vi "Merge Image Manager.vi"(7 "Calling VI Ref":refnum<vi>) -> ()   [LabVIEW 2016]
uses:
  Merge Image Type Defs/Merge Image - Image Control.ctl
  <vilib>/Utility/miscctls.llb/LVPointTypeDef.ctl
  <vilib>/vision/Image Controls.llb/IMAQ Image.ctl
  Merge Image Type Defs/Merge Image - Notifier Type.ctl
  Merge Image Type Defs/Merge Image - Actions.ctl
  Merge Image Type Defs/Merge Image - Last Used Save Type.ctl
  <vilib>/vision/NI_Vision_Development_Module.lvlib
panel:
  in  "Zero All":bool
  out "Overlay Error":errorcluster
  in  "Load":bool
  in  "Save":bool
  in  "Update Rate (ms)":i32=50
  in  "Merge Visible":bool
  in  "Hold Blue":bool
  in  "Hold Green":bool
  in  "Hold Red":bool
  in  "Blue LUT":cluster{"Blue Min (%)":i32, "Blue Max (%)":i32}={"Blue Min (%)"=0, "Blue Max (%)"=100} {"Blue Max (%)" max=100; "Blue Min (%)" max=100}
  in  "Green LUT":T1={"Green Min (%)"=0, "Green Max (%)"=100} {"Green Max (%)" max=100; "Green Min (%)" max=100}
  in  "Red LUT":cluster{"Red Min (%)":i32, "Red Max (%)":i32}={"Red Min (%)"=0, "Red Max (%)"=100} {"Red Max (%)" max=100; "Red Min (%)" max=100}
  in  "Blue Image":T2 {"Rotation (°)" format="%#.2f"; "Image" items=["None", "Image 01", "Image 02", "Merge Image"]}
  in  "Green Image":T2 {"Rotation (°)" format="%#.2f"; "Image" items=["None", "Image 01", "Image 02", "Merge Image"]}
  in  "Red Image":T2 {"Rotation (°)" format="%#.2f"; "Image" items=["None", "Image 01", "Image 02", "Merge Image"]}
  in  "Quit":bool
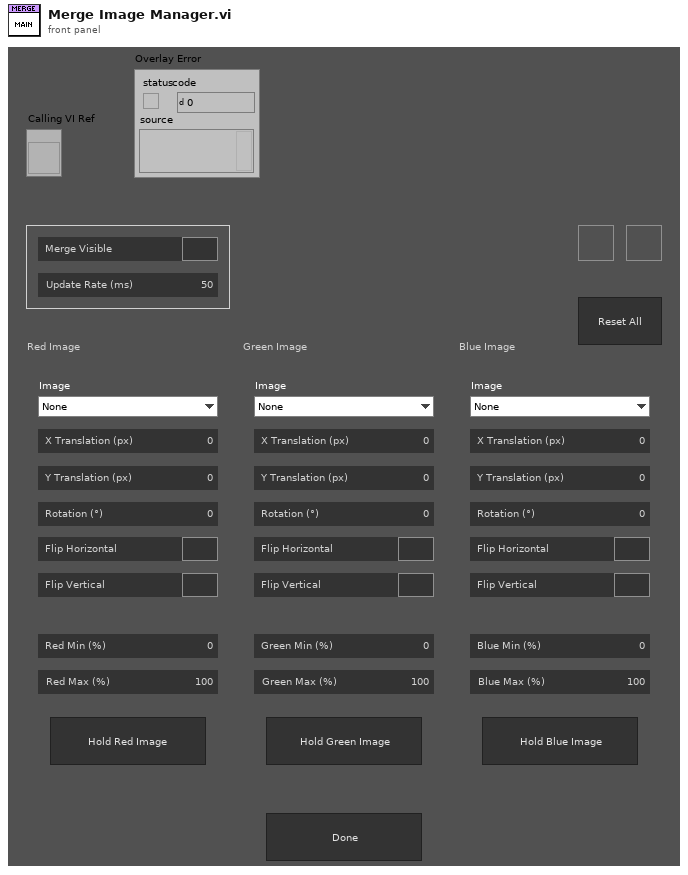
[diagram p1: front panel]
types:
  T1 = cluster{"Green Min (%)":i32, "Green Max (%)":i32}
  T2 = typedef "Merge Image - Image Control.ctl" = cluster{"Image":i32, "X Translation (px)":i32, "Y Translation (px)":i32, "Rotation (°)":sgl, "Flip Horizontal":bool, "Flip Vertical":bool}
  T3 = typedef "Merge Image - Last Used Save Type.ctl" = cluster{"Merge Contols":T2[], "LUT Controls":cluster{"Red Min (%)":i32, "Red Max (%)":i32}[]}
  T4 = typedef "Image Type" = u32
  T5 = typedef "Merge Image - Actions.ctl" = enum16{"Timeout", "Update Image Source", "Update LUTs", "Quit"}
  T6 = typedef "Merge Image - Notifier Type.ctl" = cluster{"Actions":T5, "Merge Contols":T2[], "LUT Controls":cluster{"Red Min (%)":i32, "Red Max (%)":i32}[]}
  T7 = typedef "IMAQ Image.ctl" = refnum<image>
  T8 = enum16{"Always On", "Always Off", "Off While Running"}
  T9 = typedef "LVPointTypeDef.ctl" = cluster{"Horizontal":i16, "Vertical":i16}
  T10 = typedef "LVRectTypeDef.ctl" = cluster{"Left":i16, "Top":i16, "Right":i16, "Bottom":i16}
  T11 = typedef "LVBoundsTypeDef.ctl" = cluster{"Width":u32, "Height":u32}
  T12 = enum32{"Invalid", "Standard", "Closed", "Hidden", "Minimized", "Maximized"}
  T13 = enum32{"Invalid", "Default", "Floating", "Floating/Auto-Hide", "Modal"}
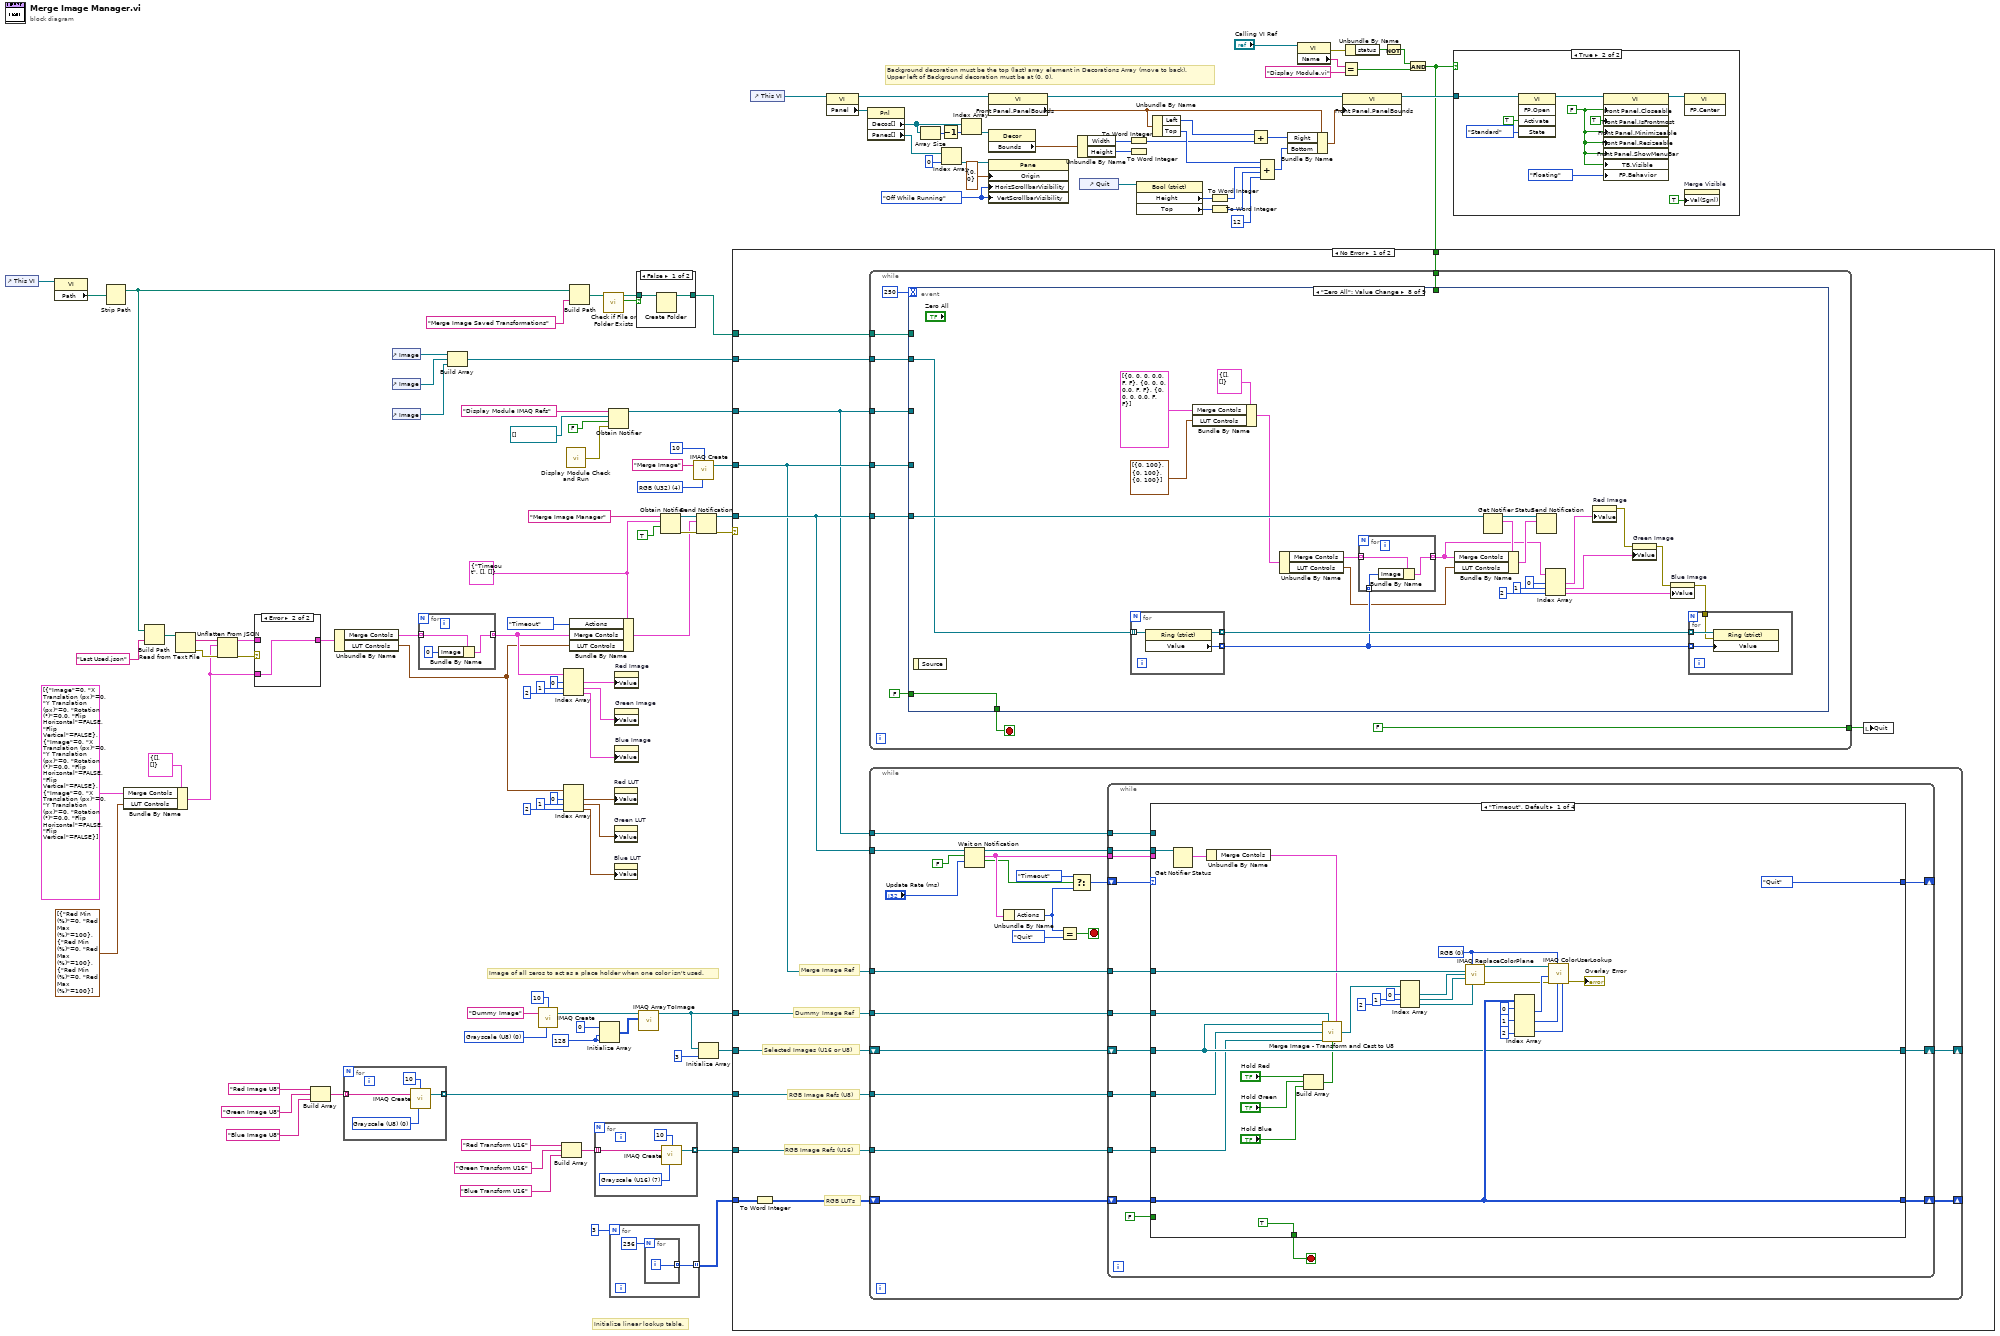
[diagram p0: block diagram]
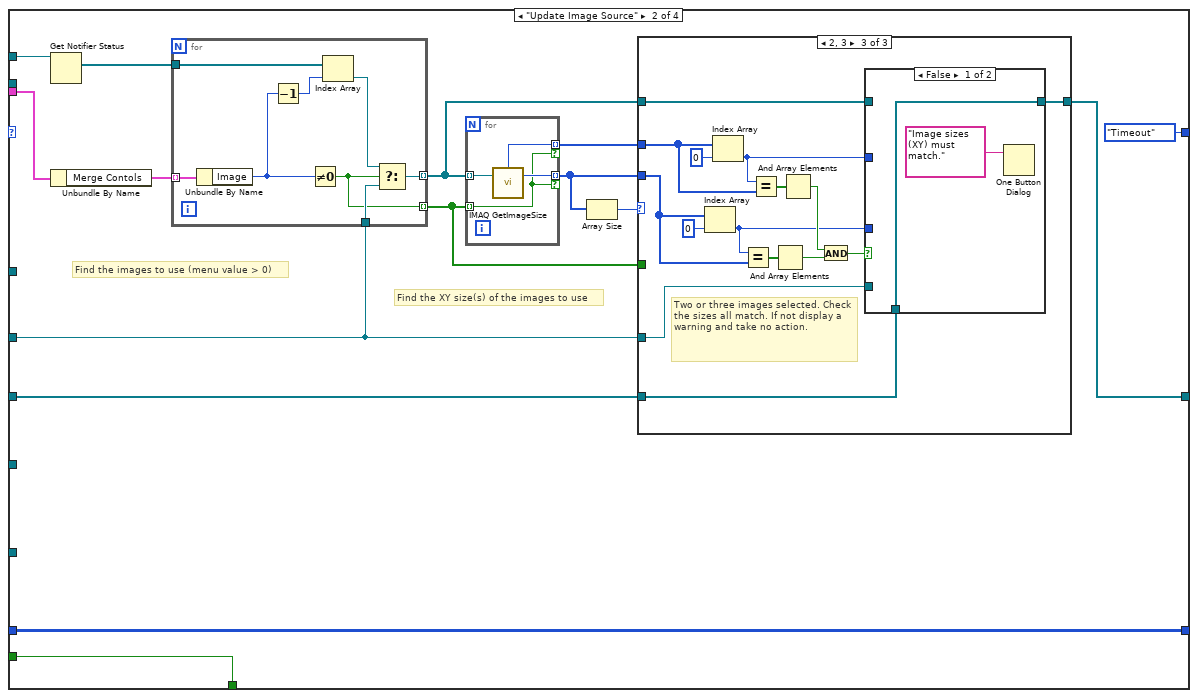
[diagram p5: hidden frame]
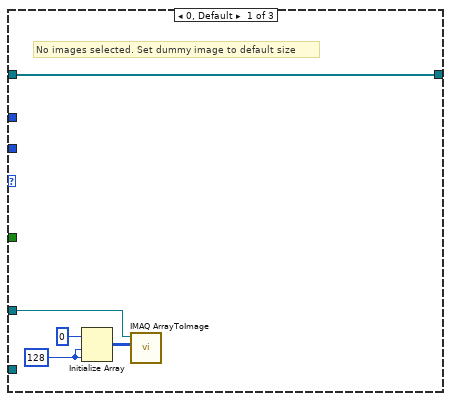
[diagram p6: hidden frame]
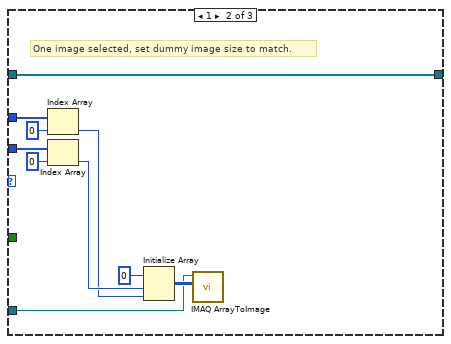
[diagram p7: hidden frame]
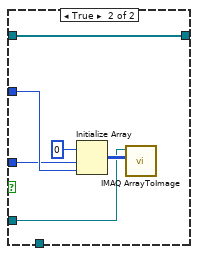
[diagram p8: hidden frame]
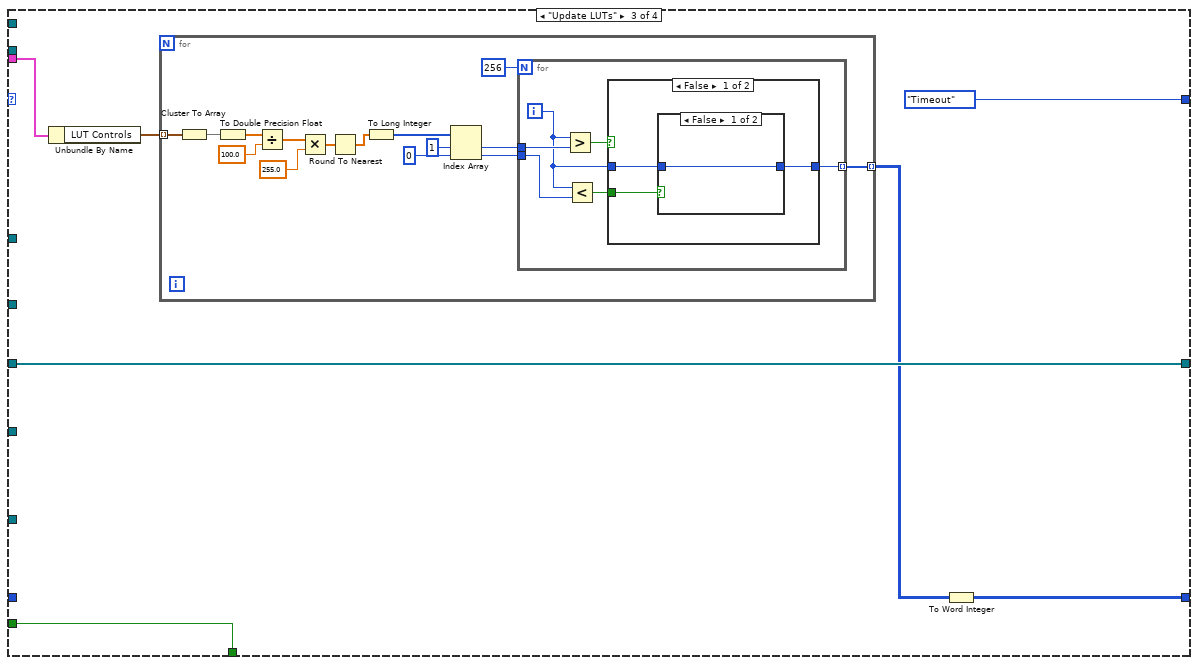
[diagram p9: hidden frame]
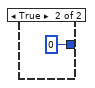
[diagram p10: hidden frame]
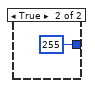
[diagram p11: hidden frame]
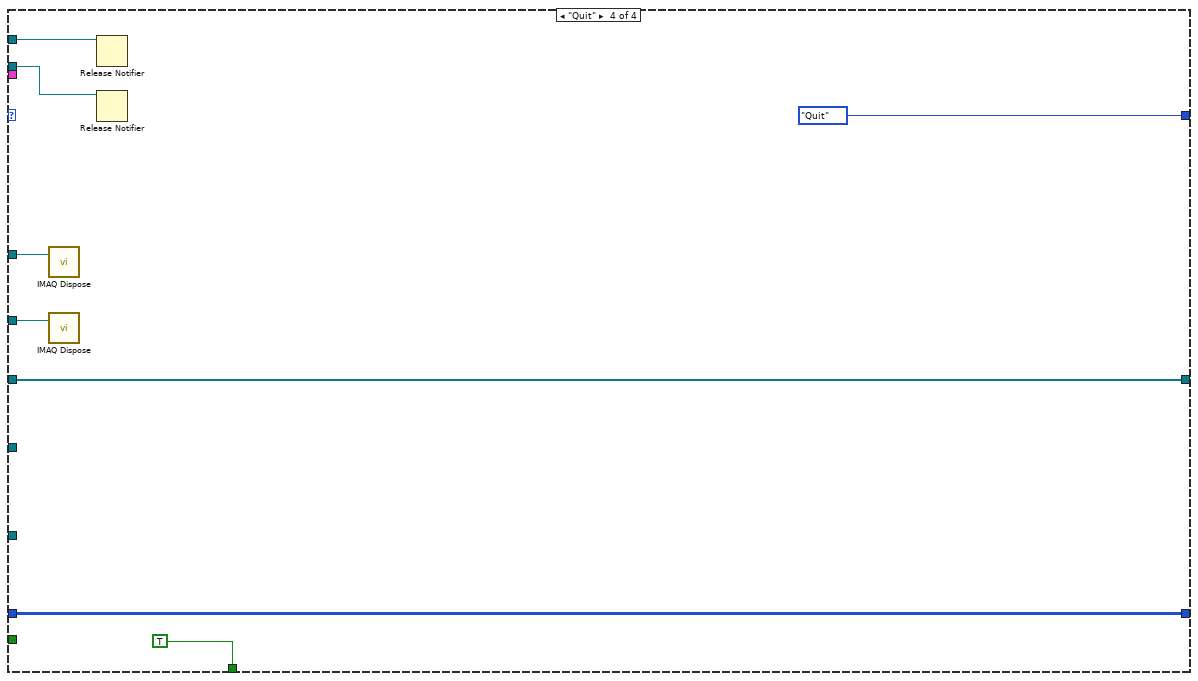
[diagram p12: hidden frame]
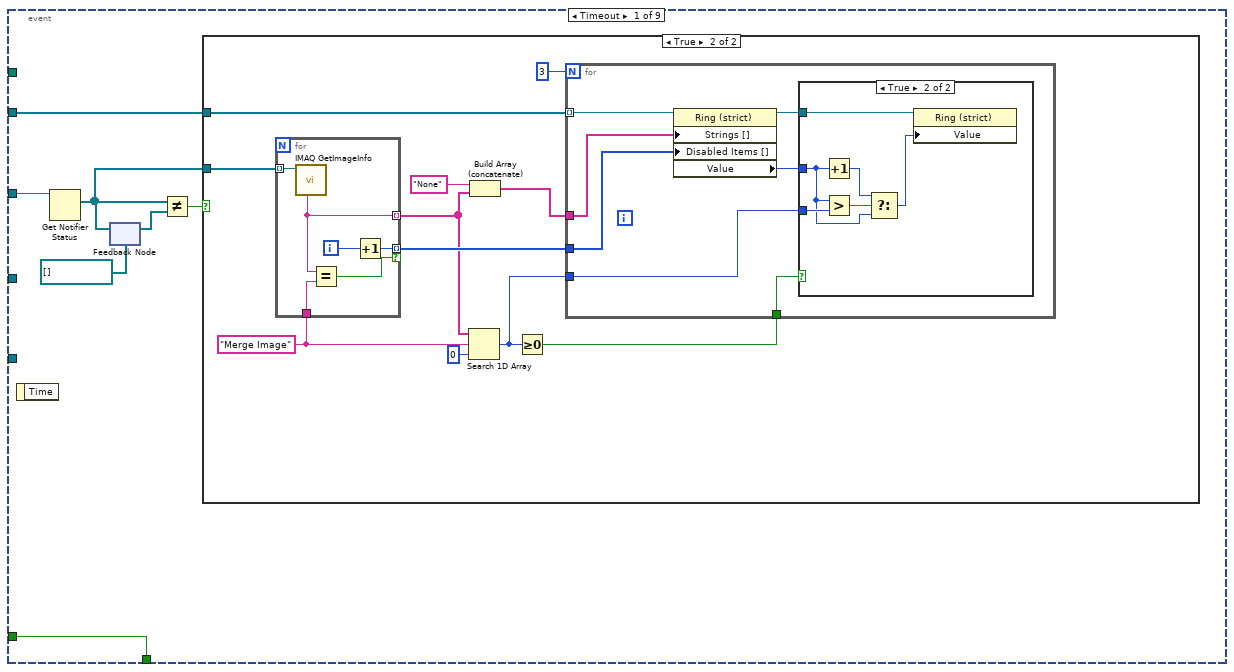
[diagram p13: hidden frame]
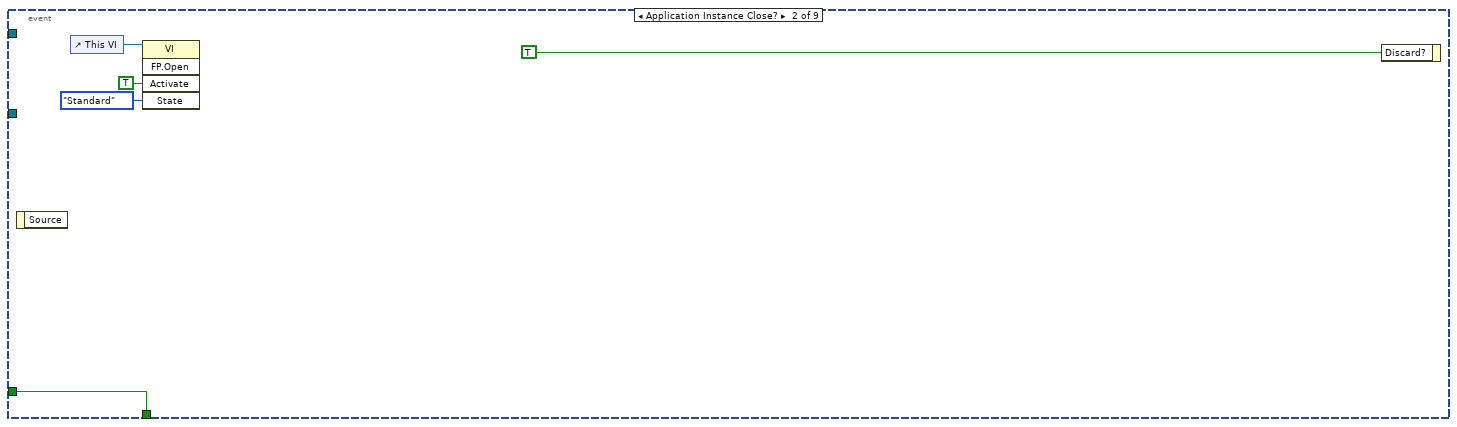
[diagram p16: hidden frame]
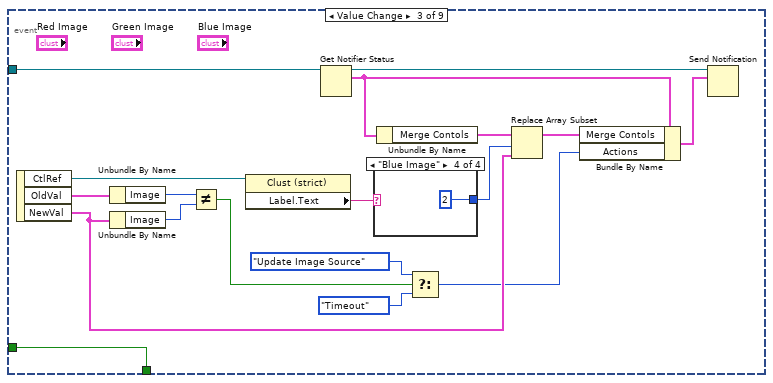
[diagram p17: hidden frame]
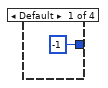
[diagram p18: hidden frame]
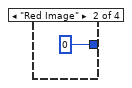
[diagram p19: hidden frame]
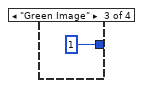
[diagram p20: hidden frame]
diagram:
  w53 = 128 ("dimension size")
  w58 = T4 0 items=["Grayscale (U8)", "Grayscale (I16)", "Grayscale (SGL)", "Complex (CSG)", "RGB (U32)", "HSL (U32)", "RGB (U64)", "Grayscale (U16)"] ("Image Type")
  w62 = T6 {"Actions"=enum."Timeout", "Merge Contols"=[], "LUT Controls"=[]} ("Merge Image Notifier Type")
  w71 = T4 4 items=["Grayscale (U8)", "Grayscale (I16)", "Grayscale (SGL)", "Complex (CSG)", "RGB (U32)", "HSL (U32)", "RGB (U64)", "Grayscale (U16)"] ("Image Type")
  w99 = T8."Off While Running" ("Vertical Scrollbar Visibility")
  # "Image of all zeros to act as a place holder when one color isn't used."
  # "Initialize linear lookup table."
  # "Background decoration must be the top (last) array element in Decorations Array (move to back).\nUpper left of Background decoration must be at (0, 0)."
  n1 = control-ref of="This VI"() -> (w83:refnum<vi>)
  n2 = property class="VI"(reference=w83) -> ("Path"=w82:path)  [unwired: 1 in, 2 out]
  n3 = Strip Path(path=w82) -> (stripped path=w26:path)  [unwired: 1 out]
  n4 = Bundle By Name(cluster=T3 {"Merge Contols"=[], "LUT Controls"=[]} ("Merge Image Last Used Type"), "Merge Contols"=T2[] [{"Image"=0, "X Translation (px)"=0, "Y Translation (px)"=0, "Rotation (°)"=0.0, "Flip Horizontal"=FALSE, "Flip Vertical"=FALSE}, {"Image"=0, "X Translation (px)"=0, "Y Translation (px)"=0, "Rotation (°)"=0.0, "Flip Horizontal"=FALSE, "Flip Vertical"=FALSE}, {"Image"=0, "X Translation (px)"=0, "Y Translation (px)"=0, "Rotation (°)"=0.0, "Flip Horizontal"=FALSE, "Flip Vertical"=FALSE}], "LUT Controls"=cluster{"Red Min (%)":i32, "Red Max (%)":i32}[] [{"Red Min (%)"=0, "Red Max (%)"=100}, {"Red Min (%)"=0, "Red Max (%)"=100}, {"Red Min (%)"=0, "Red Max (%)"=100}]) -> (w5:T3)
  n5 = Build Path(base path=w26, name or relative path="Last Used.json") -> (appended path=w25:path)
  n6 = Read from Text File(file (use dialog)=w25) -> (text=w24:string, error out=w23:errorcluster)  [unwired: 3 in, 2 out]
  n7 = Unflatten From JSON(JSON string=w24, type and defaults=w5, error in (no error)=w23) -> (value=w21:T3, error out=w22:errorcluster)  [unwired: 4 in]
  n8 = case shown="Error" w22 {
    tunnel: w21 -> [w117 _]
    tunnel: [w117 w118] -> w4
    tunnel: w5 -> [_ w118]
    frame No Error {
    }
    frame Error {
    }
  }
  n9 = Build Array("Red Image U8" ("Image Name"), "Green Image U8" ("Image Name"), "Blue Image U8" ("Image Name")) -> (w47:string[])
  n10 = Unbundle By Name(w4) -> ("Merge Contols"=w3:T2[], "LUT Controls"=w1:cluster{"Red Min (%)":i32, "Red Max (%)":i32}[])
  n11 = for {
    tunnel: w47 -> [w120] mode=indexing
    tunnel: [w119] -> w46 mode=indexing
    w121 = T4 0 items=["Grayscale (U8)", "Grayscale (I16)", "Grayscale (SGL)", "Complex (CSG)", "RGB (U32)", "HSL (U32)", "RGB (U64)", "Grayscale (U16)"] ("Image Type")
    n12 = call "IMAQ Create"("Border Size"=10, "Image Name"=w120, "Image Type"=w121) -> ("New Image"=w119:T7)  [unwired: 2 in, 1 out]
  }
  n13 = control-ref of="Image"() -> (w67:refnum<vi>)
  n14 = control-ref of="Image"() -> (w65:refnum<vi>)
  n15 = control-ref of="Image"() -> (w66:refnum<vi>)
  n16 = for {
    tunnel: w3 -> [w125] mode=indexing
    tunnel: [w123] -> w2 mode=indexing
    n17 = Bundle By Name(cluster=w125, "Image"=0) -> (w123:T2)
  }
  n18 = Build Array(w67, w65, w66) -> (w64:refnum<vi>[])
  n19 = call "IMAQ Create"("Border Size"=10, "Image Name"="Dummy Image", "Image Type"=w58) -> ("New Image"=w59:T7)  [unwired: 2 in, 1 out]
  n20 = Build Array("Red Transform U16" ("Image Name"), "Green Transform U16" ("Image Name"), "Blue Transform U16" ("Image Name")) -> (w42:string[])
  n21 = Index Array(array=w2, index #1=0 ("index"), index #2=1 ("index"), index #3=2 ("index")) -> (element #1=w17:T2, element #2=w15:T2, element #3=w16:T2)
  n22 = Index Array(array=w1, index #1=0 ("index"), index #2=1 ("index"), index #3=2 ("index")) -> (element #1=w11:cluster{"Red Min (%)":i32, "Red Max (%)":i32}, element #2=w9:cluster{"Red Min (%)":i32, "Red Max (%)":i32}, element #3=w10:cluster{"Red Min (%)":i32, "Red Max (%)":i32})
  n23 = call "Display Module Check and Run.vi"() -> ("Error"=w63:errorcluster)  [unwired: 15 in]
  n24 = Bundle By Name(cluster=w62, "Actions"=Merge_Image_-_Actions."Timeout", "Merge Contols"=w2, "LUT Controls"=w1) -> (w60:T6)
  n25 = Build Path(base path=w26, name or relative path="Merge Image Saved Transformations") -> (appended path=w80:path)
  n26 = for {
    tunnel: w42 -> [w127] mode=indexing
    tunnel: [w126] -> w38 mode=indexing
    w128 = T4 7 items=["Grayscale (U8)", "Grayscale (I16)", "Grayscale (SGL)", "Complex (CSG)", "RGB (U32)", "HSL (U32)", "RGB (U64)", "Grayscale (U16)"] ("Image Type")
    n27 = call "IMAQ Create"("Border Size"=10, "Image Name"=w127, "Image Type"=w128) -> ("New Image"=w126:T7)  [unwired: 2 in, 1 out]
  }
  n28 = Initialize Array(u8 0 ("element"), w53, w53) -> (w54:u8[][])
  n29 = call <vilib>:"Check if File or Folder Exists.vi"("path"=w80) -> ("file or folder exists?"=w79:bool, "dup path"=w78:path)  [unwired: 8 in, 1 out]
  n30 = Obtain Notifier(name (unnamed)="Display Module IMAQ Refs", notification data type=T7[] [], create if not found? (T)=FALSE, error in (no error)=w63) -> (notifier out=w68:refnum<notifier>)  [unwired: 2 out]
  n31 = for {
    N: 3 -> [_]
    tunnel: [w130] -> w51 mode=indexing
    n32 = for {
      N: 256 -> [_]
      tunnel: [w132] -> w130 mode=indexing
      i -> [w132]
    }
  }
  n33 = property on="Red LUT" class="Clust (strict)"("Value"=w11) -> ()  [unwired: 2 in, 2 out]
  n34 = property on="Green LUT" class="Clust (strict)"("Value"=w9) -> ()  [unwired: 2 in, 2 out]
  n35 = property on="Blue LUT" class="Clust (strict)"("Value"=w10) -> ()  [unwired: 2 in, 2 out]
  n36 = property on="Red Image" class="Clust (strict)"("Value"=w17) -> ()  [unwired: 2 in, 2 out]
  n37 = property on="Green Image" class="Clust (strict)"("Value"=w15) -> ()  [unwired: 2 in, 2 out]
  n38 = property on="Blue Image" class="Clust (strict)"("Value"=w16) -> ()  [unwired: 2 in, 2 out]
  n39 = case shown="False" w79 {
    tunnel: w78 -> [w134 w135]
    tunnel: [w133 w135] -> w37
    frame False {
      n40 = Create Folder(path (use dialog)=w134) -> (created path=w133:path)  [unwired: 2 in, 2 out]
    }
    frame True {
    }
  }
  n41 = call "IMAQ ArrayToImage"("Image Pixels (U8)"=w54, "Image"=w59) -> ("Image Out"=w43:T7)  [unwired: 8 in, 1 out]
  n42 = Obtain Notifier(name (unnamed)="Merge Image Manager", notification data type=w62, create if not found? (T)=TRUE) -> (notifier out=w85:refnum<notifier>, error out=w77:errorcluster)  [unwired: 1 in, 1 out]
  n43 = call "IMAQ Create"("Border Size"=10, "Image Name"="Merge Image", "Image Type"=w71) -> ("New Image"=w69:T7)  [unwired: 2 in, 1 out]
  n44 = Send Notification(notification=w60, notifier=w85, error in (no error)=w77) -> (notifier out=w84:refnum<notifier>, error out=w76:errorcluster)
  n45 = Initialize Array(w43, 3 ("dimension size")) -> (w44:T7[])
  n46 = control-ref of="This VI"() -> (w91:refnum<vi>)
  n47 = property class="VI"(reference=w91) -> (reference out=w100:refnum<vi>, "Panel"=w92:refnum<vi>)  [unwired: 1 in, 1 out]
  n48 = property class="Pnl"(reference=w92) -> ("Decos[]"=w90:refnum<vi>[], "Panes[]"=w96:refnum<vi>[])  [unwired: 1 in, 2 out]
  n49 = Array Size(array=w90) -> (size(s)=w88:i32)
  n50 = Decrement(x=w88) -> (x-1=w89:i32)
  n51 = Index Array(array=w96, index=0) -> (element=w95:refnum<vi>)
  n52 = Index Array(array=w90, index=w89) -> (element=w98:refnum<vi>)
  n53 = property class="VI"(reference=w100) -> (reference out=w102:refnum<vi>, "Front Panel.PanelBounds"=w103:T10)  [unwired: 1 in, 1 out]
  n54 = property class="Decor"(reference=w98) -> ("Bounds"=w101:T11)  [unwired: 1 in, 2 out]
  n55 = property class="Pane"(reference=w95, "Origin"=T9 {"Horizontal"=0, "Vertical"=0}, "HorizScrollbarVisibility"=w99, "VertScrollbarVisibility"=w99) -> ()  [unwired: 1 in, 2 out]
  n56 = Unbundle By Name(w101) -> ("Width"=w106:u32, "Height"=w109:u32)
  n57 = control-ref of="Quit"() -> (w93:refnum<vi>)
  n58 = To Word Integer(number=w106) -> (16bit integer=w108:i16)
  n59 = To Word Integer(number=w109) -> ()  [unwired: 1 out]
  n60 = property class="Bool (strict)"(reference=w93) -> ("Height"=w111:u32, "Top"=w112:i32)  [unwired: 1 in, 2 out]
  n61 = Unbundle By Name(w103) -> ("Left"=w105:i16, "Top"=w116:i16)
  n62 = To Word Integer(number=w111) -> (16bit integer=w114:i16)
  n63 = To Word Integer(number=w112) -> (16bit integer=w115:i16)
  n64 = Add(x=w105, y=w108) -> (x+y=w107:i16)
  n65 = Compound Arithmetic op=ADD(w116, w114, w115, i16 12 ("y")) -> (w110:i16)
  n66 = Bundle By Name(cluster=w103, "Right"=w107, "Bottom"=w110) -> (w104:T10)
  n67 = property class="VI"(reference="Calling VI Ref") -> (error out=w32:errorcluster, "Name"=w35:string)  [unwired: 1 in, 1 out]
  n68 = Equal?(x=w35, y="Display Module.vi") -> (x = y?=w29:bool)
  n69 = property class="VI"(reference=w102, "Front Panel.PanelBounds"=w104) -> (reference out=w33:refnum<vi>)  [unwired: 1 in, 1 out]
  n70 = Unbundle By Name(w32) -> ("status"=w31:bool)
  n71 = Not(x=w31) -> (.not. x?=w30:bool)
  n72 = And(x=w30, y=w29) -> (x .and. y?=w28:bool)
  n73 = case shown="No Error" w76 {
    selector: w76 -> [_ w566]
    tunnel: w84 -> [w147 w568]
    tunnel: w69 -> [w143 w567]
    tunnel: w68 -> [w142 w569]
    tunnel: w64 -> [w146 _]
    tunnel: w43 -> [w145 _]
    tunnel: w46 -> [w141 _]
    tunnel: w51 -> [w144 _]
    tunnel: w44 -> [w140 _]
    tunnel: w38 -> [w139 _]
    tunnel: w37 -> [w137 _]
    tunnel: w28 -> [w136 _]
    frame No Error {
      # "RGB Image Refs (U16)"
      # "Selected Images (U16 or U8)"
      # "Merge Image Ref"
      # "Dummy Image Ref"
      # "RGB Image Refs (U8)"
      # "RGB LUTs"
      n74 = To Word Integer(number=w144) -> (16bit integer=w138:i16[][])
      n75 = while {
        tunnel: w147 -> [w330]
        tunnel: [FALSE] -> w148
        tunnel: w143 -> [w328]
        tunnel: w142 -> [w327]
        tunnel: w146 -> [w326]
        tunnel: w137 -> [w324]
        tunnel: w136 -> [w323]
        stop <- w331 stop-if-true
        n76 = event shown="[7] \"Zero All\": Value Change" {
          selector: _ -> [_ _ _ _ _ _ _ _ _]
          dyn-events: _ -> [_ _ _ _ _ _ _ _ _]
          timeout: 250 -> [_ _ _ _ _ _ _ _ _]
          tunnel: FALSE -> [w339 w373 w392 w410 w425 w466 w484 w536 _]
          tunnel: [w339 w373 w392 w410 w425 w466 w484 w536 w562] -> w331
          tunnel: w330 -> [_ _ w391 w409 _ w465 w475 w535 w561]
          tunnel: w328 -> [_ _ _ _ w417 _ _ _ _]
          tunnel: w327 -> [w338 _ _ _ w416 _ _ _ _]
          tunnel: w326 -> [w334 _ _ _ w415 _ w472 w534 _]
          tunnel: w324 -> [_ _ _ _ _ w463 w479 _ _]
          tunnel: w323 -> [_ _ _ _ _ _ _ _ w557]
          event Timeout {
            n77 = event-data() -> ()  [unwired: 1 in, 1 out]
            n78 = Get Notifier Status(notifier=w338) -> (current notification=w333:T7[])  [unwired: 1 in, 4 out]
            n79 = feedback-in #1(w333) -> ()
            n80 = feedback #1(T7[] []) -> (w336:T7[])
            n81 = Not Equal?(x=w333, y=w336) -> (x != y?=w335:bool)
            n82 = case shown="True" w335 {
              tunnel: w334 -> [_ w349]
              tunnel: w333 -> [_ w350]
              frame False {
              }
              frame True {
                w343 = "Merge Image" ("Image Name")
                n83 = for {
                  tunnel: w350 -> [w369] mode=indexing
                  tunnel: [w368] -> w344 mode=indexing
                  tunnel: [w367] -> w345 mode=indexing if=w365
                  tunnel: w343 -> [w364]
                  i -> [w366]
                  n84 = call "IMAQ GetImageInfo"("Image"=w369) -> ("Image Name"=w368:string)  [unwired: 3 in, 7 out]
                  n85 = Equal?(x=w368, y=w364) -> (x = y?=w365:bool)
                  n86 = Increment(x=w366) -> (x+1=w367:i32)
                }
                n87 = Search 1D Array(1D array=w344, element=w343, start index (0)=0) -> (index of element=w340:i32)
                n88 = Build Array (concatenate)("None", w344) -> (w347:string[])
                n89 = Greater Or Equal To 0?(x=w340) -> (x >= 0?=w341:bool)
                n90 = for {
                  N: 3 -> [_]
                  tunnel: w349 -> [w357] mode=indexing
                  tunnel: w347 -> [w356]
                  tunnel: w345 -> [w355]
                  tunnel: w341 -> [w352]
                  tunnel: w340 -> [w351]
                  n91 = property class="Ring (strict)"(reference=w357, "Strings []"=w356, "Disabled Items []"=w355) -> (reference out=w354:refnum<vi>, "Value"=w353:i32)  [unwired: 1 in, 1 out]
                  n92 = case shown="True" w352 {
                    tunnel: w354 -> [_ w363]
                    tunnel: w353 -> [_ w358]
                    tunnel: w351 -> [_ w362]
                    frame False {
                    }
                    frame True {
                      n93 = Increment(x=w358) -> (x+1=w360:i32)
                      n94 = Greater?(x=w358, y=w362) -> (0:w361:bool)
                      n95 = Select(t=w360, s=w361, f=w358) -> (s? t:f=w359:i32)
                      n96 = property class="Ring (strict)"(reference=w363, "Value"=w359) -> ()  [unwired: 1 in, 2 out]
                    }
                  }
                }
              }
            }
          }
          event Application Instance Close? {
            n97 = event-data() -> ()  [unwired: 1 in, 1 out]
            n98 = control-ref of="This VI"() -> (w370:refnum<vi>)
            n99 = invoke class="VI" method="FP.Open"(reference=w370, "Activate"=TRUE ("Activate?"), "State"=T12."Standard") -> ()  [unwired: 2 in, 5 out]
            n100 = event-data("Discard?"=TRUE) -> ()  [unwired: 1 in, 1 out]
          }
          event Value Change {
            n101 = event-data() -> ("CtlRef"=w389:refnum<vi>, "OldVal"=w382:T2, "NewVal"=w379:T2)  [unwired: 1 in]
            n102 = Unbundle By Name(w382) -> ("Image"=w381:i32)
            n103 = Unbundle By Name(w379) -> ("Image"=w380:i32)
            n104 = Not Equal?(x=w381, y=w380) -> (x != y?=w378:bool)
            n105 = property class="Clust (strict)"(reference=w389) -> ("Label.Text"=w388:string)  [unwired: 1 in, 2 out]
            n106 = Get Notifier Status(notifier=w391) -> (notifier out=w390:refnum<notifier>, current notification=w383:T6)  [unwired: 1 in, 3 out]
            n107 = case shown="\"Blue Image\"" w388 {
              tunnel: [-1 0 1 2] -> w386
              frame Default {
              }
              frame "Red Image" {
              }
              frame "Green Image" {
              }
              frame "Blue Image" {
              }
            }
            n108 = Unbundle By Name(w383) -> ("Merge Contols"=w387:T2[])
            n109 = Select(t=Merge_Image_-_Actions."Update Image Source" ("Actions"), s=w378, f=Merge_Image_-_Actions."Timeout" ("Actions")) -> (s? t:f=w375:T5)
            n110 = Replace Array Subset(array=w387, new element=w379, index=w386) -> (w385:T2[])
            n111 = Bundle By Name(cluster=w383, "Merge Contols"=w385, "Actions"=w375) -> (w384:T6)
            n112 = Send Notification(notification=w384, notifier=w390) -> ()  [unwired: 1 in, 2 out]
          }
          event "Red LUT", "Green LUT", "Blue LUT": Value Change {
            n113 = event-data() -> ("NewVal"=w399:variant, "CtlRef"=w400:refnum<vi>)  [unwired: 1 in]
            n114 = Variant To Data(type=cluster{"Red Min (%)":u16, "Red Max (%)":u16} {"Red Min (%)"=0, "Red Max (%)"=100} ("LUT Controls"), Variant=w399) -> (data=w397:cluster{"Red Min (%)":u16, "Red Max (%)":u16})  [unwired: 1 in, 1 out]
            n115 = property class="Clust (strict)"(reference=w400) -> ("Label.Text"=w407:string)  [unwired: 1 in, 2 out]
            n116 = Get Notifier Status(notifier=w409) -> (notifier out=w408:refnum<notifier>, current notification=w401:T6)  [unwired: 1 in, 3 out]
            n117 = case shown="\"Red LUT\"" w407 {
              tunnel: [-1 0 1 2] -> w405
              frame Default {
              }
              frame "Red LUT" {
              }
              frame "Green LUT" {
              }
              frame "Blue LUT" {
              }
            }
            n118 = Unbundle By Name(w401) -> ("LUT Controls"=w406:cluster{"Red Min (%)":i32, "Red Max (%)":i32}[])
            n119 = Replace Array Subset(array=w406, new element=w397, index=w405) -> (w404:cluster{"Red Min (%)":i32, "Red Max (%)":i32}[])
            n120 = Bundle By Name(cluster=w401, "Actions"=Merge_Image_-_Actions."Update LUTs", "LUT Controls"=w404) -> (w402:T6)
            n121 = Send Notification(notification=w402, notifier=w408) -> ()  [unwired: 1 in, 2 out]
          }
          event "Merge Visible": Value Change {
            n122 = event-data() -> ("NewVal"=w418:bool)  [unwired: 1 in]
            n123 = Get Notifier Status(notifier=w416) -> (notifier out=w424:refnum<notifier>, current notification=w422:T7[], error out=w423:errorcluster)  [unwired: 1 in, 2 out]
            n124 = case shown="False" w418 {
              tunnel: w424 -> [w434 w451]
              tunnel: w423 -> [w432 w450]
              tunnel: w422 -> [w431 w449]
              tunnel: [w433 w447] -> w419
              tunnel: [w434 w451] -> w421
              tunnel: [w432 w450] -> w420
              tunnel: w417 -> [w430 w448]
              tunnel: w415 -> [w427 _]
              frame False {
                n125 = Search 1D Array(1D array=w431, element=w430, start index (0)=0) -> (index of element=w426:i32)
                n126 = Greater Or Equal To 0?(x=w426) -> (x >= 0?=w428:bool)
                n127 = case shown="True" w428 {
                  tunnel: w426 -> [_ w445]
                  tunnel: w431 -> [w442 w444]
                  tunnel: [w442 w443] -> w433
                  frame False {
                  }
                  frame True {
                    n128 = Delete From Array(array=w444, length=1, index=w445) -> (array with subset deleted=w443:T7[])  [unwired: 1 out]
                  }
                }
                n129 = for {
                  tunnel: w427 -> [w441] mode=indexing
                  tunnel: w426 -> [w439]
                  n130 = property class="Ring (strict)"(reference=w441) -> (reference out=w440:refnum<vi>, "Value"=w435:i32)  [unwired: 1 in, 1 out]
                  n131 = Greater?(x=w435, y=w439) -> (0:w438:bool)
                  n132 = Decrement(x=w435) -> (x-1=w437:i32)
                  n133 = Select(t=w437, s=w438, f=w435) -> (s? t:f=w436:i32)
                  n134 = property class="Ring (strict)"(reference=w440, "Value"=w436) -> ()  [unwired: 1 in, 2 out]
                }
              }
              frame True {
                n135 = Build Array (concatenate)(w449, w448) -> (w447:T7[])
              }
            }
            n136 = Send Notification(notification=w419, notifier=w421, error in (no error)=w420) -> ()  [unwired: 2 out]
          }
          event "Save": Value Change {
            n137 = event-data() -> ()  [unwired: 1 in, 1 out]
            n138 = Get Notifier Status(notifier=w465) -> (current notification=w464:T6)  [unwired: 1 in, 4 out]
            n139 = Unbundle By Name(w464) -> ("Merge Contols"=w454:T2[], "LUT Controls"=w453:cluster{"Red Min (%)":i32, "Red Max (%)":i32}[])
            n140 = Bundle By Name(cluster=T3 {"Merge Contols"=[], "LUT Controls"=[]} ("Merge Image Last Used Type"), "Merge Contols"=w454, "LUT Controls"=w453) -> (w452:T3)
            n141 = Flatten To JSON(anything=w452) -> (JSON string=w457:string, 11:w456:errorcluster)  [unwired: 2 in]
            n142 = call "File Dialog"("start path"=w463, "prompt"="Save Transformation Parameters", "error in"=w456, "pattern (all files)"="*.json", "pattern label"="JSON") -> ("selected path"=w458:path, "error out"=w459:errorcluster)  [unwired: 7 in, 2 out]
            n143 = case shown="No Error" w459 {
              tunnel: w458 -> [w468 _]
              tunnel: w457 -> [w467 _]
              frame No Error {
                n144 = Write to Text File(file (use dialog)=w468, text=w467) -> ()  [unwired: 2 in, 3 out]
              }
              frame Error {
              }
            }
          }
          event "Load": Value Change {
            n145 = event-data() -> ()  [unwired: 1 in, 1 out]
            n146 = call "File Dialog2"("start path"=w479, "prompt"="Load Transformation Parameters", "pattern (all files)"="*.json", "pattern label"="JSON") -> ("selected path"=w480:path, "error out"=w478:errorcluster)  [unwired: 8 in, 2 out]
            n147 = for {
              tunnel: w472 -> [w487] mode=indexing
              tunnel: [w486] -> w470 mode=indexing
              tunnel: [w485] -> w471 mode=indexing
              n148 = property class="Ring (strict)"(reference=w487) -> (reference out=w485:refnum<vi>, "Value"=w486:i32)  [unwired: 1 in, 1 out]
            }
            n149 = Read from Text File(file (use dialog)=w480, error in=w478) -> (text=w477:string, error out=w476:errorcluster)  [unwired: 2 in, 2 out]
            n150 = Unflatten From JSON(JSON string=w477, type and defaults=T3 {"Merge Contols"=[], "LUT Controls"=[]} ("Merge Image Last Used Type"), error in (no error)=w476) -> (value=w474:T3, error out=w473:errorcluster)  [unwired: 4 in]
            n151 = case shown="No Error" w473 {
              tunnel: w475 -> [w506 _]
              tunnel: w474 -> [w492 _]
              tunnel: w471 -> [w496 _]
              tunnel: w470 -> [w488 _]
              frame No Error {
                n152 = Unbundle By Name(w492) -> ("Merge Contols"=w491:T2[], "LUT Controls"=w490:cluster{"Red Min (%)":i32, "Red Max (%)":i32}[])
                n153 = for {
                  tunnel: w491 -> [w509] mode=indexing
                  tunnel: [w508] -> w489 mode=indexing
                  tunnel: w488 -> [w507] mode=indexing
                  n154 = Bundle By Name(cluster=w509, "Image"=w507) -> (w508:T2)
                }
                n155 = Get Notifier Status(notifier=w506) -> (notifier out=w505:refnum<notifier>, current notification=w504:T6)  [unwired: 1 in, 3 out]
                n156 = Bundle By Name(cluster=w504, "Merge Contols"=w489, "LUT Controls"=w490) -> (w503:T6)
                n157 = Send Notification(notification=w503, notifier=w505) -> ()  [unwired: 1 in, 2 out]
                n158 = Index Array(array=w489, index #1=0 ("index"), index #2=1 ("index"), index #3=2 ("index")) -> (element #1=w499:T2, element #2=w498:T2, element #3=w497:T2)
                n159 = property on="Red Image" class="Clust (strict)"("Value"=w499) -> (error out=w495:errorcluster)  [unwired: 2 in, 1 out]
                n160 = property on="Green Image" class="Clust (strict)"(error in=w495, "Value"=w498) -> (error out=w494:errorcluster)  [unwired: 1 in, 1 out]
                n161 = property on="Blue Image" class="Clust (strict)"(error in=w494, "Value"=w497) -> (error out=w493:errorcluster)  [unwired: 1 in, 1 out]
                n162 = for {
                  tunnel: w496 -> [w512] mode=indexing
                  tunnel: w488 -> [w511] mode=indexing
                  tunnel: w493 -> [w510]
                  n163 = property class="Ring (strict)"(reference=w512, error in=w510, "Value"=w511) -> ()  [unwired: 2 out]
                }
              }
              frame Error {
              }
            }
          }
          event "Zero All": Value Change {
            n164 = event-data() -> ()  [unwired: 1 in, 1 out]
            n165 = for {
              tunnel: w534 -> [w545] mode=indexing
              tunnel: [w544] -> w532 mode=indexing
              tunnel: [w543] -> w533 mode=indexing
              n166 = property class="Ring (strict)"(reference=w545) -> (reference out=w543:refnum<vi>, "Value"=w544:i32)  [unwired: 1 in, 1 out]
            }
            n167 = Bundle By Name(cluster=T3 {"Merge Contols"=[], "LUT Controls"=[]} ("Merge Image Last Used Type"), "Merge Contols"=T2[] [{"Image"=0, "X Translation (px)"=0, "Y Translation (px)"=0, "Rotation (°)"=0.0, "Flip Horizontal"=FALSE, "Flip Vertical"=FALSE}, {"Image"=0, "X Translation (px)"=0, "Y Translation (px)"=0, "Rotation (°)"=0.0, "Flip Horizontal"=FALSE, "Flip Vertical"=FALSE}, {"Image"=0, "X Translation (px)"=0, "Y Translation (px)"=0, "Rotation (°)"=0.0, "Flip Horizontal"=FALSE, "Flip Vertical"=FALSE}], "LUT Controls"=cluster{"Red Min (%)":i32, "Red Max (%)":i32}[] [{"Red Min (%)"=0, "Red Max (%)"=100}, {"Red Min (%)"=0, "Red Max (%)"=100}, {"Red Min (%)"=0, "Red Max (%)"=100}]) -> (w513:T3)
            n168 = Unbundle By Name(w513) -> ("Merge Contols"=w519:T2[], "LUT Controls"=w518:cluster{"Red Min (%)":i32, "Red Max (%)":i32}[])
            n169 = for {
              tunnel: w519 -> [w539] mode=indexing
              tunnel: [w538] -> w517 mode=indexing
              tunnel: w532 -> [w537] mode=indexing
              n170 = Bundle By Name(cluster=w539, "Image"=w537) -> (w538:T2)
            }
            n171 = Get Notifier Status(notifier=w535) -> (notifier out=w531:refnum<notifier>, current notification=w530:T6)  [unwired: 1 in, 3 out]
            n172 = Bundle By Name(cluster=w530, "Merge Contols"=w517, "LUT Controls"=w518) -> (w529:T6)
            n173 = Send Notification(notification=w529, notifier=w531) -> ()  [unwired: 1 in, 2 out]
            n174 = Index Array(array=w517, index #1=0 ("index"), index #2=1 ("index"), index #3=2 ("index")) -> (element #1=w525:T2, element #2=w524:T2, element #3=w523:T2)
            n175 = property on="Red Image" class="Clust (strict)"("Value"=w525) -> (error out=w522:errorcluster)  [unwired: 2 in, 1 out]
            n176 = property on="Green Image" class="Clust (strict)"(error in=w522, "Value"=w524) -> (error out=w521:errorcluster)  [unwired: 1 in, 1 out]
            n177 = property on="Blue Image" class="Clust (strict)"(error in=w521, "Value"=w523) -> (error out=w520:errorcluster)  [unwired: 1 in, 1 out]
            n178 = for {
              tunnel: w533 -> [w542] mode=indexing
              tunnel: w532 -> [w541] mode=indexing
              tunnel: w520 -> [w540]
              n179 = property class="Ring (strict)"(reference=w542, error in=w540, "Value"=w541) -> ()  [unwired: 2 out]
            }
          }
          event "Quit": Value Change {
            n180 = event-data() -> ("NewVal"=w562:bool)  [unwired: 1 in]
            n181 = Get Notifier Status(notifier=w561) -> (notifier out=w560:refnum<notifier>, current notification=w551:T6)  [unwired: 1 in, 3 out]
            n182 = control-ref of="This VI"() -> (w556:refnum<vi>)
            n183 = Bundle By Name(cluster=w551, "Actions"=Merge_Image_-_Actions."Quit") -> (w558:T6)
            n184 = property class="VI"(reference=w556) -> ("Path"=w555:path)  [unwired: 1 in, 2 out]
            n185 = Unbundle By Name(w551) -> ("Merge Contols"=w548:T2[], "LUT Controls"=w547:cluster{"Red Min (%)":i32, "Red Max (%)":i32}[])
            n186 = Send Notification(notification=w558, notifier=w560) -> ()  [unwired: 1 in, 2 out]
            n187 = Strip Path(path=w555) -> (stripped path=w554:path)  [unwired: 1 out]
            n188 = Build Path(base path=w554, name or relative path="Last Used.json") -> (appended path=w552:path)
            n189 = Bundle By Name(cluster=T3 {"Merge Contols"=[], "LUT Controls"=[]} ("Merge Image Last Used Type"), "Merge Contols"=w548, "LUT Controls"=w547) -> (w546:T3)
            n190 = Flatten To JSON(anything=w546) -> (JSON string=w550:string)  [unwired: 2 in, 1 out]
            n191 = Write to Text File(file (use dialog)=w552, text=w550) -> ()  [unwired: 2 in, 3 out]
            n192 = case shown="True" w557 {
              frame False {
              }
              frame True {
                n193 = control-ref of="This VI"() -> (w563:refnum<vi>)
                n194 = invoke class="VI" method="FP.Close"(reference=w563) -> ()  [unwired: 2 in, 3 out]
              }
            }
          }
        }
      }
      n195 = while {
        tunnel: w147 -> [w168]
        tunnel: w145 -> [w158]
        shift-right: [w155] -> _
        shift-left: w140 -> [w157]
        shift-right: [w154] -> _
        shift-left: w138 -> [w156]
        tunnel: w143 -> [w153]
        tunnel: w142 -> [w152]
        tunnel: w141 -> [w151]
        tunnel: w139 -> [w150]
        stop <- w166 stop-if-true
        n196 = Wait on Notification(notifier=w168, ignore previous (F)=FALSE, timeout in ms (-1)="Update Rate (ms)") -> (notifier out=w164:refnum<notifier>, notification=w165:T6, timed out?=w162:bool)  [unwired: 1 in, 1 out]
        n197 = Unbundle By Name(w165) -> ("Actions"=w161:T5)
        n198 = Equal?(x=w161, y=Merge_Image_-_Actions."Quit") -> (x = y?=w166:bool)
        n199 = Select(t=Merge_Image_-_Actions."Timeout", s=w162, f=w161) -> (s? t:f=w159:T5)
        n200 = while {
          shift-right: [w181] -> _
          shift-left: w159 -> [w183]
          tunnel: w165 -> [w182]
          tunnel: w164 -> [w180]
          tunnel: w158 -> [w177]
          tunnel: w153 -> [w171]
          tunnel: w152 -> [w172]
          shift-right: [w174] -> w155
          shift-left: w157 -> [w176]
          tunnel: w151 -> [w170]
          tunnel: w150 -> [w169]
          shift-right: [w173] -> w154
          shift-left: w156 -> [w175]
          stop <- w178 stop-if-true
          n201 = case shown="\"Timeout\", Default" w183 {
            tunnel: w182 -> [_ w227 w284 _]
            tunnel: [Merge_Image_-_Actions."Quit" ("y") Merge_Image_-_Actions."Timeout" ("y") Merge_Image_-_Actions."Timeout" ("y") Merge_Image_-_Actions."Quit" ("y")] -> w181
            tunnel: w180 -> [w185 _ _ w316]
            tunnel: FALSE -> [_ w230 w286 _]
            tunnel: [TRUE w230 w286 TRUE] -> w178
            tunnel: w177 -> [w209 w216 _ w320]
            tunnel: w176 -> [w212 w217 w285 w318]
            tunnel: w175 -> [w213 w228 _ w319]
            tunnel: [w212 w218 w285 w318] -> w174
            tunnel: [w213 w228 w281 w319] -> w173
            tunnel: w172 -> [_ w225 _ w315]
            tunnel: w171 -> [w214 _ _ w317]
            tunnel: w170 -> [w211 _ _ _]
            tunnel: w169 -> [w210 _ _ _]
            frame "Timeout", Default {
              w199 = u16 0 items=["RGB", "HSL", "HSV", "HSI"] ("Color Mode")
              n202 = Get Notifier Status(notifier=w185) -> (current notification=w184:T6)  [unwired: 1 in, 4 out]
              n203 = Unbundle By Name(w184) -> ("Merge Contols"=w208:T2[])
              n204 = Build Array("Hold Red", "Hold Green", "Hold Blue") -> (w187:bool[])
              n205 = call "Merge Image - Transform and Cast to U8.vi"("Selected Image (U8 or U16)"=w212, "Dummy Image Ref"=w209, "Transform Parameters"=w208, "RGB Image Refs (U8)"=w211, "RGB Image Refs (U16)"=w210, "Image Holds"=w187) -> ("RGB Image Refs (U8 DUP)"=w207:T7[])  [unwired: 9 in]
              n206 = Index Array(array=w207, index #1=0 ("index"), index #2=1 ("index"), index #3=2 ("index")) -> (element #1=w203:T7, element #2=w202:T7, element #3=w201:T7)
              n207 = call "IMAQ ReplaceColorPlane"("Color Mode"=w199, "Image Dst"=w214, "Red or Hue Plane"=w203, "Green or Sat Plane"=w202, "Blue or Luma or Val or Inten Plane"=w201) -> ("Image Dst Out"=w192:T7, "error out"=w191:errorcluster)  [unwired: 9 in]
              n208 = Index Array(array=w213, index (row) #1=0 ("index (row)"), index (row) #2=1 ("index (row)"), index (row) #3=2 ("index (row)")) -> (element #1=w195:i16[], element #2=w194:i16[], element #3=w193:i16[])  [unwired: 3 in]
              n209 = call "IMAQ ColorUserLookup"("Blue or Luma or Val or Inten Lookup Table"=w193, "Green or Sat Lookup Table"=w194, "Color Mode"=w199, "error in (no error)"=w191, "Red or Hue Lookup Table"=w195, "Image Src"=w192) -> ("error out"=→"Overlay Error":errorcluster)  [unwired: 4 in, 1 out]
            }
            frame "Update Image Source" {
              # "Find the XY size(s) of the images to use"
              # "Find the images to use (menu value > 0)"
              n210 = Get Notifier Status(notifier=w225) -> (current notification=w224:T7[])  [unwired: 1 in, 4 out]
              n211 = Unbundle By Name(w227) -> ("Merge Contols"=w226:T2[])
              n212 = for {
                tunnel: w226 -> [w280] mode=indexing
                tunnel: w224 -> [w279]
                tunnel: [w275] -> w219 mode=indexing
                tunnel: w216 -> [w274]
                tunnel: [w273] -> w220 mode=indexing
                n213 = Unbundle By Name(w280) -> ("Image"=w278:i32)
                n214 = Decrement(x=w278) -> (x-1=w277:i32)
                n215 = Not Equal To 0?(x=w278) -> (x != 0?=w273:bool)
                n216 = Index Array(array=w279, index=w277) -> (element=w276:T7)
                n217 = Select(t=w276, s=w273, f=w274) -> (s? t:f=w275:T7)
              }
              n218 = for {
                tunnel: w219 -> [w272] mode=indexing
                tunnel: w220 -> [w269] mode=indexing
                tunnel: [w271] -> w222 mode=indexing if=w269
                tunnel: [w270] -> w221 mode=indexing if=w269
                n219 = call "IMAQ GetImageSize"("Image"=w272) -> ("Y Resolution"=w270:i32, "X Resolution"=w271:i32)  [unwired: 3 in, 1 out]
              }
              n220 = Array Size(array=w221) -> (size(s)=w223:i32)
              n221 = case shown="2, 3" w223 {
                tunnel: w222 -> [_ w245 w255]
                tunnel: w221 -> [_ w242 w258]
                tunnel: w220 -> [_ _ _]
                tunnel: w219 -> [w232 w237 w249]
                tunnel: [w232 w237 w248] -> w218
                tunnel: w217 -> [_ _ w247]
                tunnel: w216 -> [w231 w236 w246]
                frame 0, Default {
                  w234 = 128 ("dimension size")
                  # "No images selected. Set dummy image to default size"
                  n222 = Initialize Array(u8 0 ("element"), w234, w234) -> (w233:u8[][])
                  n223 = call "IMAQ ArrayToImage"("Image Pixels (U8)"=w233, "Image"=w231) -> ()  [unwired: 8 in, 2 out]
                }
                frame 1 {
                  # "One image selected, set dummy image size to match."
                  n224 = Index Array(array=w245, index=0) -> (element=w238:i32)
                  n225 = Index Array(array=w242, index=0) -> (element=w239:i32)
                  n226 = Initialize Array(u8 0 ("element"), w239, w238) -> (w240:u8[][])
                  n227 = call "IMAQ ArrayToImage"("Image Pixels (U8)"=w240, "Image"=w236) -> ()  [unwired: 8 in, 2 out]
                }
                frame 2, 3 {
                  # "Two or three images selected. Check the sizes all match. If not display a warning and take no action."
                  n228 = Index Array(array=w258, index=0) -> (element=w250:i32)
                  n229 = Index Array(array=w255, index=0) -> (element=w251:i32)
                  n230 = Equal?(x=w250, y=w258) -> (x = y?=w257:bool[])
                  n231 = Equal?(x=w251, y=w255) -> (x = y?=w256:bool[])
                  n232 = And Array Elements(Boolean array=w257) -> (logical AND=w253:bool)
                  n233 = And Array Elements(Boolean array=w256) -> (logical AND=w254:bool)
                  n234 = And(x=w254, y=w253) -> (x .and. y?=w252:bool)
                  n235 = case shown="False" w252 {
                    tunnel: w251 -> [_ w265]
                    tunnel: w250 -> [_ w264]
                    tunnel: w249 -> [_ w268]
                    tunnel: [w262 w268] -> w248
                    tunnel: w246 -> [_ w263]
                    tunnel: w247 -> [w262 _]
                    frame False {
                      n236 = One Button Dialog(message="Image sizes (XY) must match.") -> ()  [unwired: 1 in, 1 out]
                    }
                    frame True {
                      n237 = Initialize Array(u8 0 ("element"), w264, w265) -> (w266:u8[][])
                      n238 = call "IMAQ ArrayToImage"("Image Pixels (U8)"=w266, "Image"=w263) -> ()  [unwired: 8 in, 2 out]
                    }
                  }
                }
              }
            }
            frame "Update LUTs" {
              n239 = Unbundle By Name(w284) -> ("LUT Controls"=w283:cluster{"Red Min (%)":i32, "Red Max (%)":i32}[])
              n240 = for {
                tunnel: w283 -> [w302] mode=indexing
                tunnel: [w298] -> w282 mode=indexing
                n241 = Cluster To Array(cluster=w302) -> (array=w297:i32[])
                n242 = To Double Precision Float(number=w297) -> (double precision float=w296:dbl[])
                n243 = Divide(x=w296, y=100.0) -> (x/y=w294:dbl[])
                n244 = Multiply(x=w294, y=255.0) -> (x*y=w292:dbl[])
                n245 = Round To Nearest(number=w292) -> (nearest integer value=w290:dbl[])
                n246 = To Long Integer(number=w290) -> (32bit integer=w291:i32[])
                n247 = Index Array(array=w291, index #1=1 ("index"), index #2=0 ("index")) -> (element #1=w289:i32, element #2=w288:i32)
                n248 = for {
                  N: 256 -> [_]
                  tunnel: w289 -> [w308]
                  tunnel: w288 -> [w306]
                  tunnel: [w303] -> w298 mode=indexing
                  i -> [w304]
                  n249 = Greater?(x=w304, y=w308) -> (0:w307:bool)
                  n250 = Less?(x=w304, y=w306) -> (x < y?=w305:bool)
                  n251 = case shown="False" w307 {
                    tunnel: w305 -> [w311 _]
                    tunnel: w304 -> [w310 _]
                    tunnel: [w309 255] -> w303
                    frame False {
                      n252 = case shown="False" w311 {
                        tunnel: w310 -> [w312 _]
                        tunnel: [w312 0] -> w309
                        frame False {
                        }
                        frame True {
                        }
                      }
                    }
                    frame True {
                    }
                  }
                }
              }
              n253 = To Word Integer(number=w282) -> (16bit integer=w281:i16[][])
            }
            frame "Quit" {
              n254 = call "IMAQ Dispose"("Image"=w317) -> ()  [unwired: 5 in, 1 out]
              n255 = call "IMAQ Dispose"("Image"=w320) -> ()  [unwired: 5 in, 1 out]
              n256 = Release Notifier(notifier=w315) -> ()  [unwired: 2 in, 3 out]
              n257 = Release Notifier(notifier=w316) -> ()  [unwired: 2 in, 3 out]
            }
          }
        }
      }
      n258 = local write "Quit"(w148) -> ()
    }
    frame Error {
      n259 = Release Notifier(notifier=w568, error in (no error)=w566) -> (error out=w565:errorcluster)  [unwired: 1 in, 2 out]
      n260 = call "IMAQ Dispose"("Image"=w567, "error in (no error)"=w565) -> ("error out"=w564:errorcluster)  [unwired: 4 in]
      n261 = Release Notifier(notifier=w569, error in (no error)=w564) -> ()  [unwired: 1 in, 3 out]
    }
  }
  n262 = case shown="True" w28 {
    tunnel: w33 -> [_ w577]
    frame False {
    }
    frame True {
      w572 = FALSE ("Front Panel Window:Closeable")
      n263 = invoke class="VI" method="FP.Open"(reference=w577, "Activate"=TRUE ("Activate?"), "State"=T12."Standard") -> (reference out=w576:refnum<vi>)  [unwired: 2 in, 4 out]
      n264 = property class="VI"(reference=w576, "Front Panel.Closeable"=w572, "Front Panel.IsFrontmost"=TRUE ("Front Panel Window:Is Frontmost"), "Front Panel.Minimizeable"=w572, "Front Panel.Resizeable"=w572, "Front Panel.ShowMenuBar"=w572, "TB.Visible"=w572, "FP.Behavior"=T13."Floating" ("Front Panel Window:Behavior")) -> (reference out=w573:refnum<vi>)  [unwired: 1 in, 1 out]
      n265 = property on="Merge Visible" class="Bool (strict)"("Val(Sgnl)"=TRUE ("Value (Signaling)")) -> ()  [unwired: 2 in, 2 out]
      n266 = invoke class="VI" method="FP.Center"(reference=w573) -> ()  [unwired: 2 in, 3 out]
    }
  }
